vi "Moyenne.vi"(10 "Numérique":dbl, 11 "tableau":dbl[](array[numeric])) -> (3 "mean":dbl caption="moyenne" format="%0.2f")   [LabVIEW 2017]
uses:
  <vilib>/Analysis/baseanly.llb/Mean (DBL).vi
  <vilib>/Analysis/NI_AALBase.lvlib
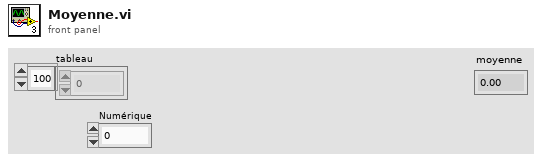
[diagram p1: front panel]
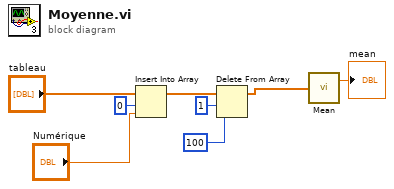
[diagram p0: block diagram]
diagram:
  n1 = Insert Into Array(array="tableau", index=0 ("indice"), new element="Numérique") -> (w6:dbl[])
  n2 = Delete From Array(array=w6, length=1 ("longueur"), index=100 ("indice")) -> (array with subset deleted=w3:dbl[])  [unwired: 1 out]
  n3 = call-poly <vilib>:"Mean.vi"("X"=w3) -> ("mean"=→"mean":dbl)  [unwired: 1 out]
